vi "INIT_path.vi"(8 "error in (no error)":errorcluster caption="错误输入（无错误）", 11 "Ignote coefficient 输入":refnum<class "Coefficient.lvclass">) -> (0 "error out":errorcluster caption="错误输出", 3 "Ignote coefficient 输出":refnum<class "Coefficient.lvclass">)   [LabVIEW 2025, in "Coefficient.lvclass"]
uses:
  Coefficient.lvclass
  Coefficient.lvclass/Coefficient.ctl
panel:
  # "现在是子类了喔"
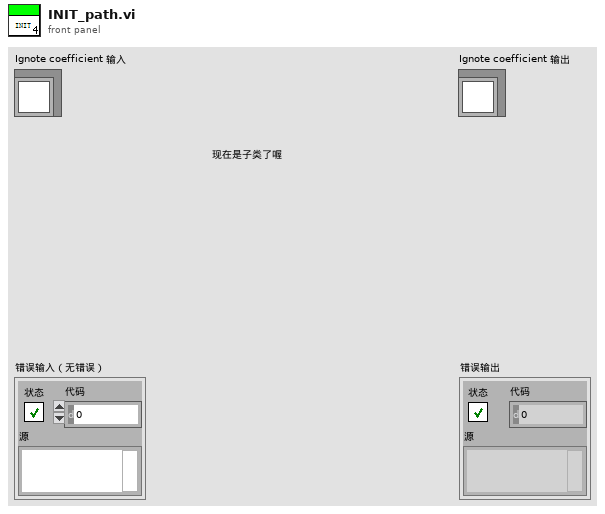
[diagram p1: front panel]
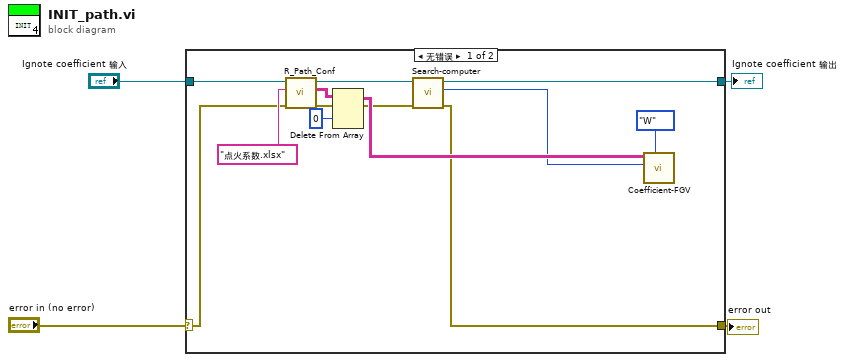
[diagram p0: block diagram]
diagram:
  n1 = case shown="无错误" "error in (no error)" {
    selector: "error in (no error)" -> [w7 w18]
    tunnel: [w6 w18] -> w3
    tunnel: [w9 w17] -> w2
    tunnel: "Ignote coefficient 输入" -> [w11 w17]
    frame No Error {
      n2 = call-dynamic "R_Path_Conf.vi"("error in (no error)"=w7, "pattern"="点火系数.xlsx", "Path_management 输入"=w11) -> ("error out"=w8:errorcluster, "data"=w15:string[][], "Path_management 输出"=w10:refnum<class "Coefficient.lvclass">)  [unwired: 6 in]
      n3 = Delete From Array(array=w15, index (row)=0 ("索引 (行)")) -> (array with subset deleted=w13:string[][])  [unwired: 2 in, 1 out]
      n4 = call-dynamic "Search-computer.vi"("error in (no error)"=w8, "Ignote coefficient 输入"=w10) -> ("error out"=w6:errorcluster, "数值"=w5:i32, "Ignote coefficient 输出"=w9:refnum<class "Coefficient.lvclass">)  [unwired: 7 in]
      n5 = call "Coefficient-FGV.vi"("枚举"=enum16{"R", "W"}."W", "机台"=w5, "dataIN"=w13) -> ()  [unwired: 7 in, 2 out]
    }
    frame Error {
    }
  }
  "error out" <- w3
  "Ignote coefficient 输出" <- w2
